vi "Read Config File Ref.vi"(8 "error in (no error)":errorcluster, 11 "Configuration File In":refnum<class "Configuration File.lvclass">) -> (0 "error out":errorcluster, 2 "refnum out":T1, 3 "Configuration File Out":refnum<class "Configuration File.lvclass">)   [LabVIEW 2020, in "Configuration File.lvclass"]
doc: "For the configuration file interface to work, the class implementing the interface needs to save the reference to the file in the class attributes. This is an accessor for that attribute which must be implemented by the class."
uses:
  Configuration File.lvclass
  C:/Git/astemes-triarc-framework/source/Framework/Configuration/Configuration.lvclass
  <vilib>/Utility/config.llb/Config Data RefNum.ctl
  Base/Base.lvclass
  <vilib>/Utility/config.llb/NI_LVConfig.lvlib
  Configuration/Configuration.lvclass
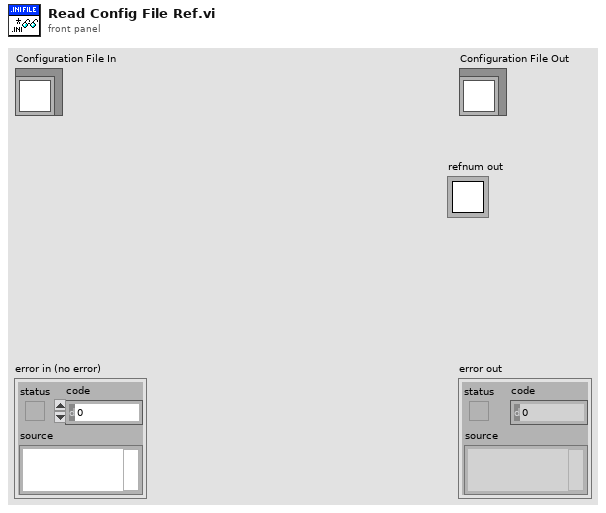
[diagram p1: front panel]
types:
  T1 = typedef "NI_LVConfig.lvlib/Config Data RefNum.ctl" = refnum<k1>
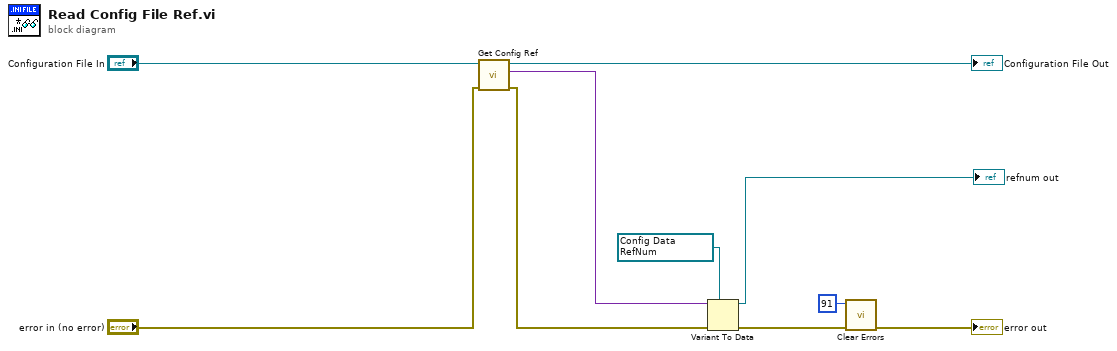
[diagram p0: block diagram]
diagram:
  w5 = T1 refnum items=["config data"] ("refnum out")
  n1 = call "Get Config Ref.vi"("error in (no error)"="error in (no error)", "Configuration In"="Configuration File In") -> ("error out"=w6:errorcluster, "Reference"=w8:variant, "Configuration Out"=→"Configuration File Out":refnum<class "Configuration File.lvclass">)  [unwired: 7 in]
  n2 = Variant To Data(error in=w6, type=w5, Variant=w8) -> (data=→"refnum out":T1, error out=w4:errorcluster)
  n3 = call <vilib>:"Clear Errors.vi"("error in (no error)"=w4, "specific error code to clear (0: all)"=91) -> ("error out"=→"error out":errorcluster)  [unwired: 4 in, 1 out]
